vi "Own20261012_SetArrayDimensions.vi"() -> ()   [LabVIEW 2024]
panel:
  out "error out":errorcluster caption="错误输出"
  in  "dimensions":u32
  in  "array_id":u32
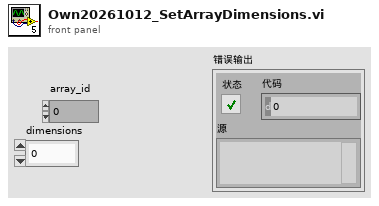
[diagram p1: front panel]
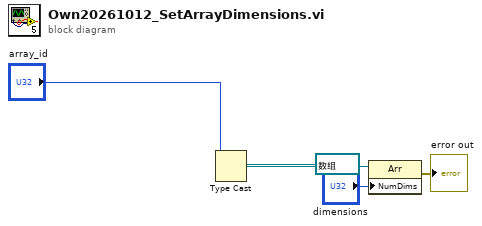
[diagram p0: block diagram]
diagram:
  n1 = Type Cast(type=refnum<vi> refnum ("引用"), x="array_id") -> (*(type *) &x=w3:refnum<vi>)
  n2 = property class="Arr"(reference=w3, "NumDims"="dimensions") -> (error out=→"error out":errorcluster)  [unwired: 1 in, 1 out]
